vi "CreateListener.vi"(8 "error in (no error)":errorcluster, 10 "service name":string, 11 "TCPIP in":refnum<class "TCPIP.lvclass">) -> (0 "error out":errorcluster, 3 "TCPIP out":refnum<class "TCPIP.lvclass">)   [LabVIEW 2018, in "TCPIP.lvclass"]
uses:
  TCPIP.lvclass
  TCPIP.lvclass/TCPIP.ctl
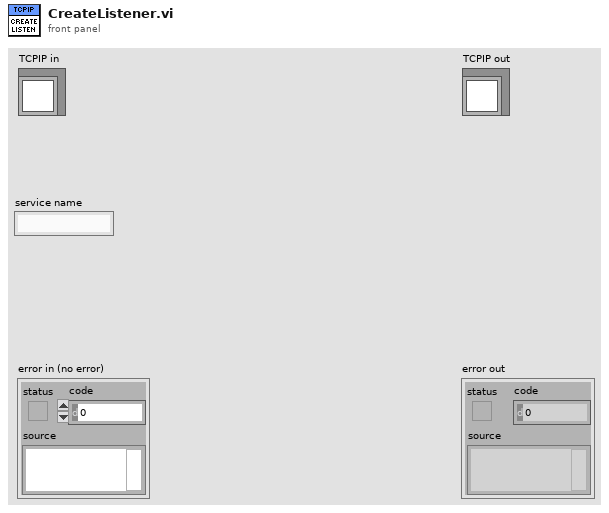
[diagram p1: front panel]
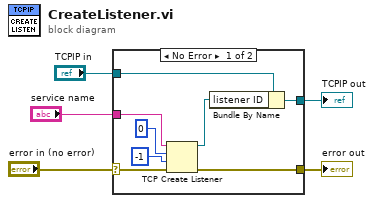
[diagram p0: block diagram]
diagram:
  n1 = case shown="No Error" "error in (no error)" {
    selector: "error in (no error)" -> [w10 w15]
    tunnel: [w9 w15] -> w4
    tunnel: [w12 w14] -> w2
    tunnel: "TCPIP in" -> [w13 w14]
    tunnel: "service name" -> [w8 _]
    frame No Error {
      n2 = TCP Create Listener(8:w10, 9:-1 ("timeout"), 10:u16 0 ("port"), 11:w8) -> (0:w9:errorcluster, 3:w11:refnum<k5>)  [unwired: 1 in, 1 out]
      n3 = Bundle By Name(cluster=w13, "listener ID"=w11) -> (w12:refnum<class "TCPIP.lvclass">)
    }
    frame Error {
    }
  }
  "error out" <- w4
  "TCPIP out" <- w2
